vi "Pre Launch Init.vi"(11 "ZM-ROOT-root in":refnum<class "ZM-ROOT-root.lvclass">) -> (0 "error out":errorcluster, 3 "ZM-ROOT-root out":refnum<class "ZM-ROOT-root.lvclass">)   [LabVIEW 2020, in "ZM-ROOT-root.lvlib" / "ZM-ROOT-root.lvclass"]
doc: "Pre Launch Init override of the root: Call Parent, then ZM-ROOT-createResources creates the stop and error user events. If that fails, what was created is destroyed and the error fails the launch. The children are launched in Actor Core, not here."
uses:
  ZM-ROOT-root.lvclass
  <vilib>/ActorFramework/Actor/Actor.lvclass
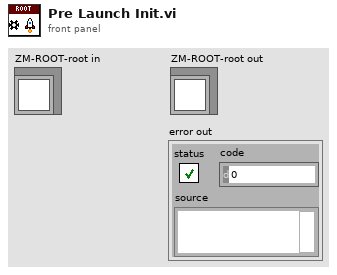
[diagram p1: front panel]
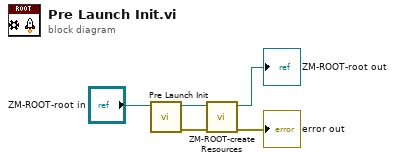
[diagram p0: block diagram]
diagram:
  n1 = call-parent "Pre Launch Init.vi"("Actor in"="ZM-ROOT-root in") -> ("error out"=w1:errorcluster, "Actor out"=w3:refnum<class "ZM-ROOT-root.lvclass">)  [unwired: 9 in]
  n2 = call "ZM-ROOT-createResources.vi"("error in (no error)"=w1, "ZM-ROOT-root in"=w3) -> ("error out"=→"error out":errorcluster, "ZM-ROOT-root out"=→"ZM-ROOT-root out":refnum<class "ZM-ROOT-root.lvclass">)  [unwired: 8 in]
